vi "Calculate Center.vi"(8 "Type of Assembly Tray":i32, 9 "Syringe Coordinates":dbl[](array[numeric]), 10 "Relative Coordinates":dbl[][](array[numeric]), 11 "Fiducial Measurements":dbl[][](array[numeric])) -> (3 "XYZTheta Centers":dbl[][](array[numeric]) format="%#.9g")   [LabVIEW 2021, in "Assembly Tray.lvclass"]
uses:
  Assembly Tray.lvclass
  <vilib>/Analysis/NI_AALPro.lvlib
  <vilib>/Analysis/coordinate.llb/2D Cartesian Coordinate Rotation (Scalar).vi
panel:
  out "gantry vs OGP XY":dbl[][][](array[numeric])
  out "actual rotation":dbl[](array[numeric])
  out "Fitted relative XY coordinates":dbl[][][](array[numeric]) format="%#.6g"
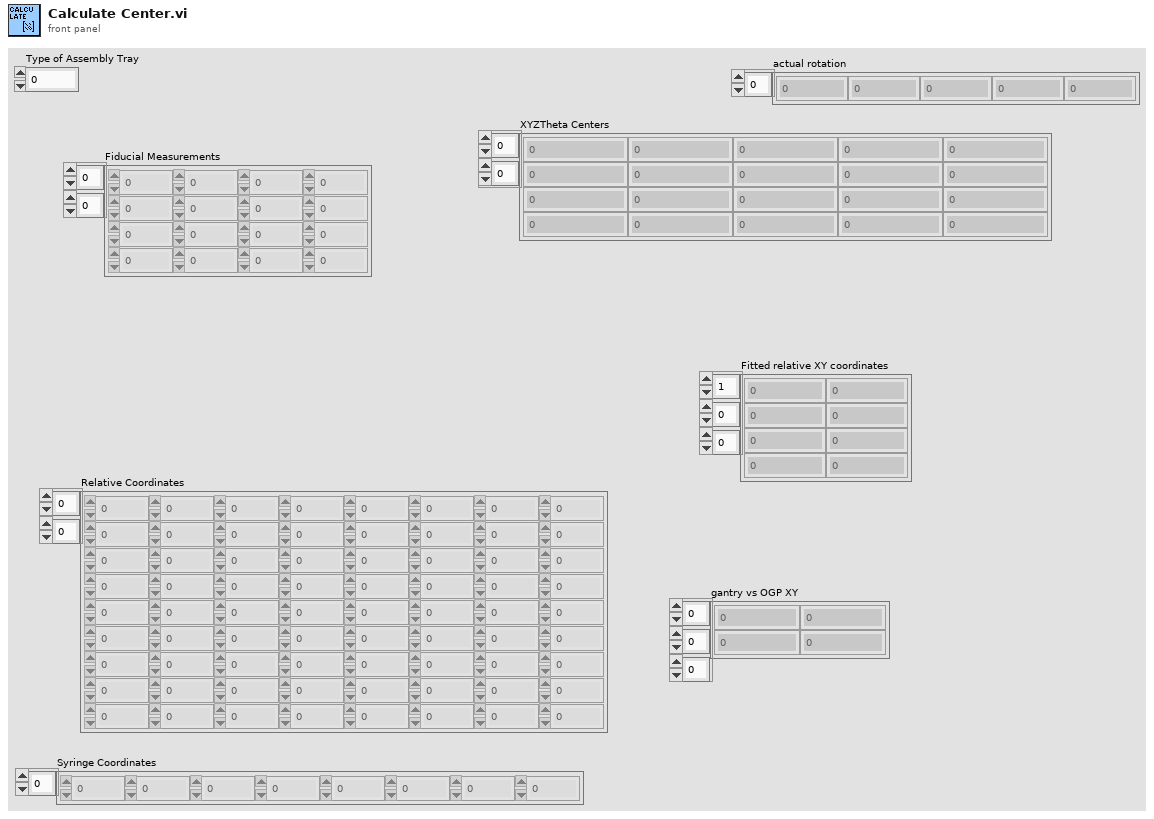
[diagram p1: front panel]
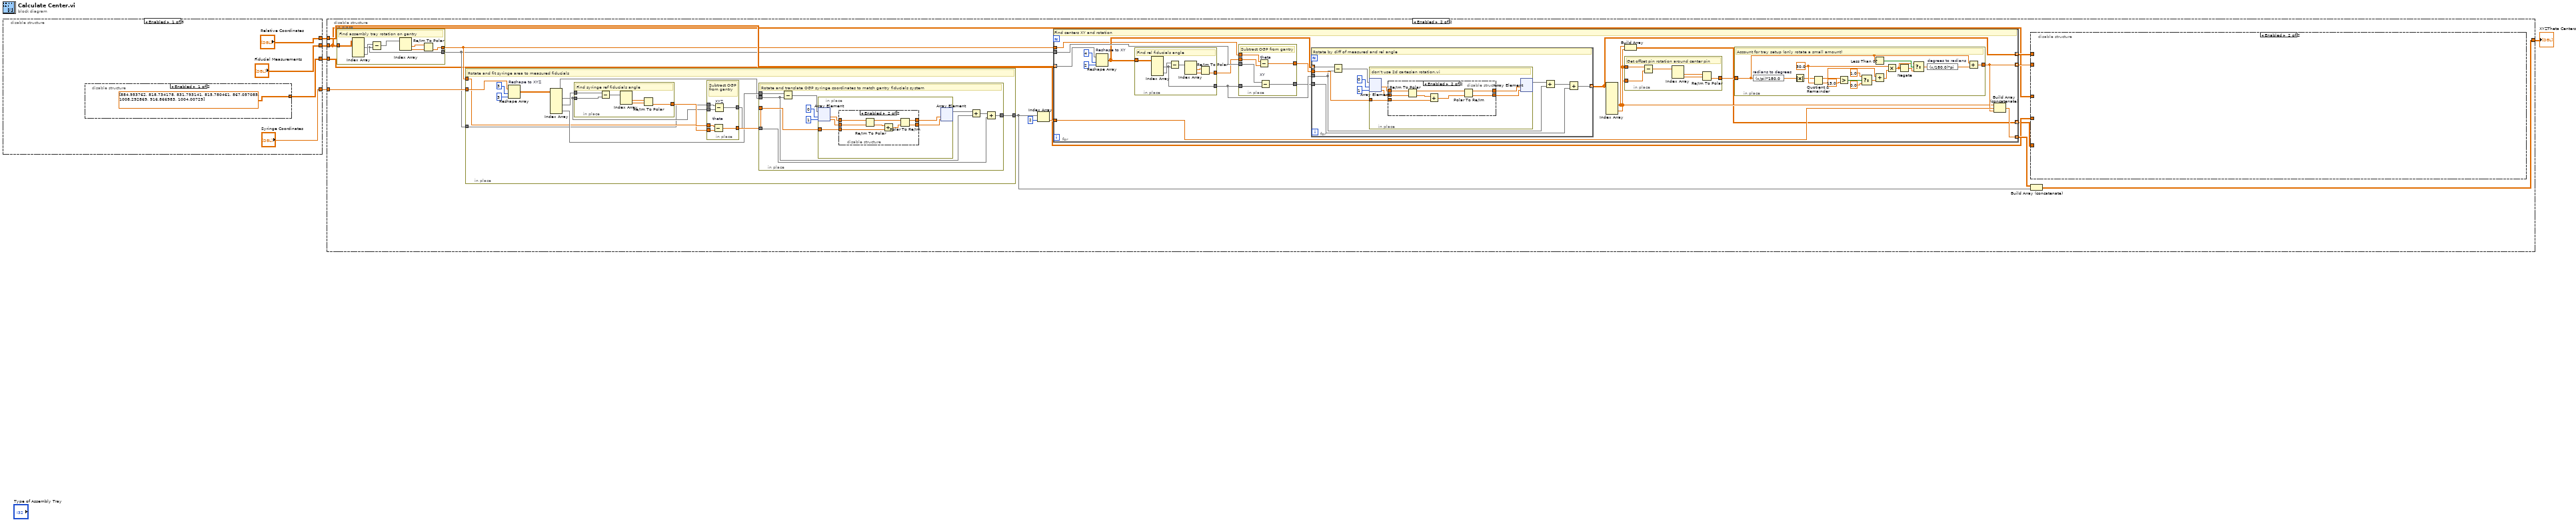
[diagram p0: block diagram]
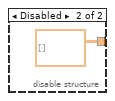
[diagram p2: hidden frame]
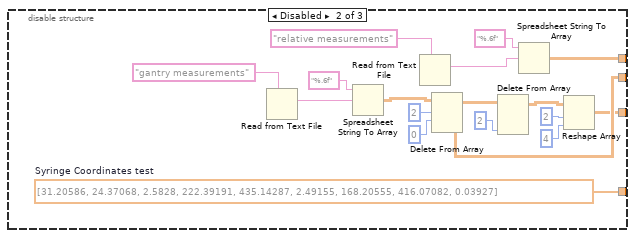
[diagram p3: hidden frame]
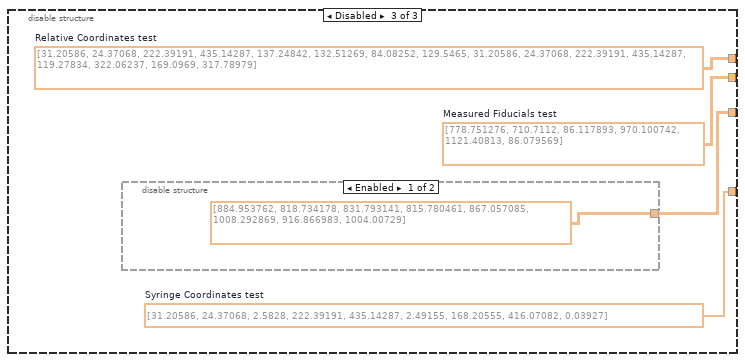
[diagram p4: hidden frame]
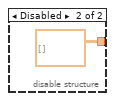
[diagram p5: hidden frame]
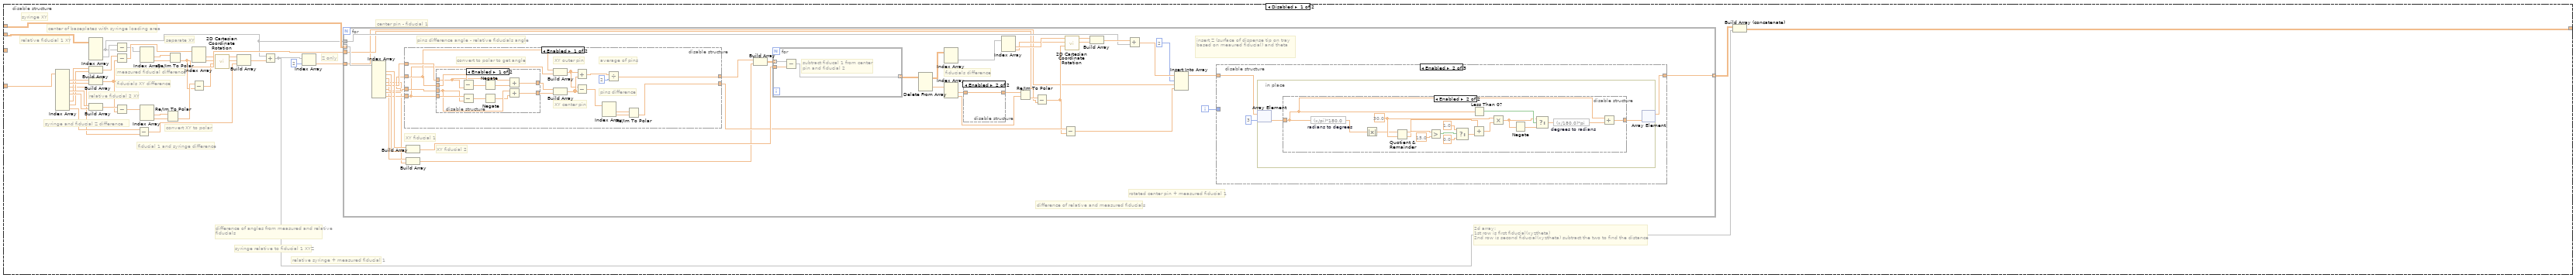
[diagram p6: hidden frame]
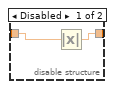
[diagram p7: hidden frame]
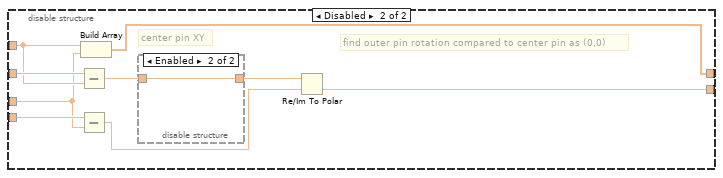
[diagram p9: hidden frame]
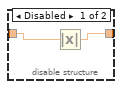
[diagram p10: hidden frame]
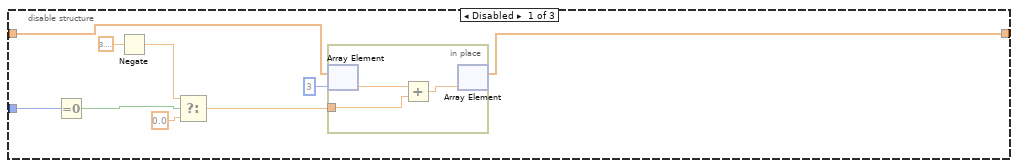
[diagram p11: hidden frame]
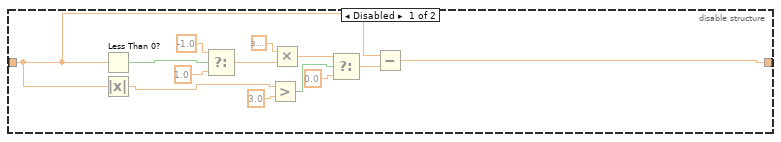
[diagram p12: hidden frame]
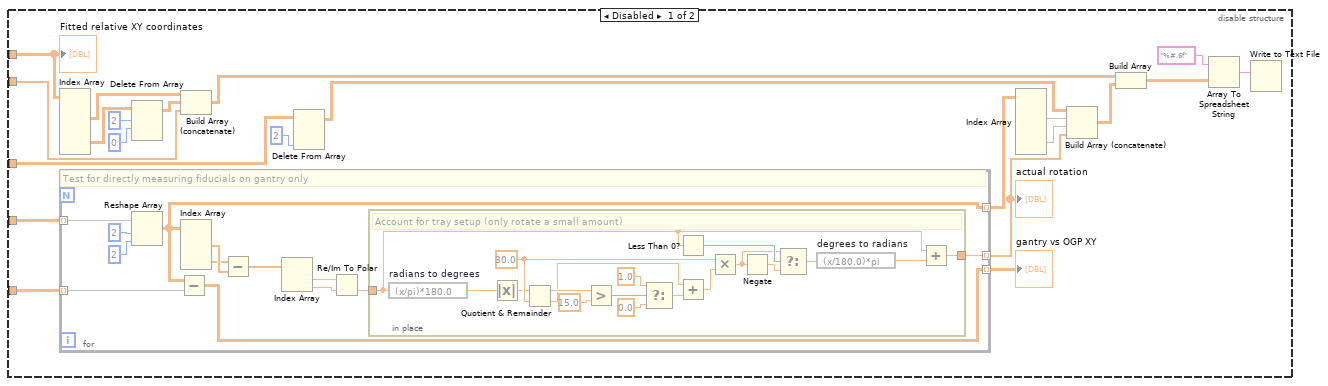
[diagram p14: hidden frame]
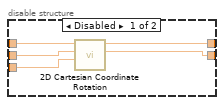
[diagram p15: hidden frame]
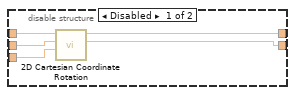
[diagram p16: hidden frame]
diagram:
  n1 = disable-structure shown="Enabled" {
    disable-tunnel: ["Syringe Coordinates" w29 w31] -> w2
    disable-tunnel: ["Fiducial Measurements" w19 w32] -> w3
    disable-tunnel: ["Relative Coordinates" w20 w33] -> w4
    disable-tunnel: [w6 w14 w30] -> w1
    frame Enabled {
      n2 = disable-structure shown="Enabled" {
        disable-tunnel: [dbl[][] [[884.953762, 818.734178, 831.793141, 815.780461], [867.057085, 1008.292869, 916.866983, 1004.00729]] dbl[][] []] -> w6
        frame Enabled {
        }
        frame Disabled {
        }
      }
    }
    frame Disabled {
      w29 = dbl[] [31.20586, 24.37068, 2.5828, 222.39191, 435.14287, 2.49155, 168.20555, 416.07082, 0.03927]  # Syringe Coordinates test
      n3 = Read from Text File(prompt (Open existing file)="gantry measurements") -> (text=w28:string)  [unwired: 3 in, 3 out]
      n4 = Spreadsheet String To Array(format string="%.6f", spreadsheet string=w28) -> (array=w12:dbl[][])  [unwired: 2 in]
      n5 = Read from Text File(prompt (Open existing file)="relative measurements") -> (text=w23:string)  [unwired: 3 in, 3 out]
      n6 = Delete From Array(array=w12, length=2, index (row)=0) -> (deleted portion=w19:dbl[][], array with subset deleted=w13:dbl[][])  [unwired: 1 in]
      n7 = Delete From Array(array=w13, index (col)=2 ("disabled index (col)")) -> (array with subset deleted=w17:dbl[][])  [unwired: 2 in, 1 out]
      n8 = Spreadsheet String To Array(format string="%.6f", spreadsheet string=w23) -> (array=w20:dbl[][])  [unwired: 2 in]
      n9 = Reshape Array(w17, 2 ("dimension size"), 4 ("dimension size")) -> (w14:dbl[][])
    }
    frame Disabled {
      w31 = dbl[] [31.20586, 24.37068, 2.5828, 222.39191, 435.14287, 2.49155, 168.20555, 416.07082, 0.03927]  # Syringe Coordinates test
      w32 = dbl[][] [[778.751276, 710.7112, 86.117893], [970.100742, 1121.40813, 86.079569]]  # Measured Fiducials test
      w33 = dbl[][] [[31.20586, 24.37068, 222.39191, 435.14287, 137.24842, 132.51269, 84.08252, 129.5465], [31.20586, 24.37068, 222.39191, 435.14287, 119.27834, 322.06237, 169.0969, 317.78979]]  # Relative Coordinates test
      n10 = disable-structure shown="Enabled" {
        disable-tunnel: [dbl[][] [[884.953762, 818.734178, 831.793141, 815.780461], [867.057085, 1008.292869, 916.866983, 1004.00729]] dbl[][] []] -> w30
        frame Enabled {
        }
        frame Disabled {
        }
      }
    }
  }
  n11 = disable-structure shown="Enabled" {
    disable-tunnel: w4 -> [w72 w217]
    disable-tunnel: w3 -> [w69 w206]
    disable-tunnel: w2 -> [w68 w216]
    disable-tunnel: [w44 w210] -> w5
    disable-tunnel: w1 -> [_ w209]
    frame Disabled {
      # "center of baseplates with syringe loading area"
      # "relative fiducial 2 XY"
      # "relative fiducial 1 XY"
      # "syringe XY"
      # "center pin - fiducial 1"
      # "Z only"
      # "relative syringe + measured fiducial 1"
      # "syringe relative to fiducial 1 XYZ"
      # "difference of angles from measured and relative fiducials"
      # "separate XY"
      # "convert XY to polar"
      # "measured fiducial difference"
      # "fiducial 1 and syringe difference"
      # "syringe and fiducial Z difference"
      # "fiducials XY difference"
      # "2d array:\n1st row is first fiducial(xyztheta)\n2nd row is second fiducial(xyztheta) subtract the two to find the distance"
      n12 = Index Array(array=w68) -> (element #1=w67:dbl, element #2=w66:dbl, element #3=w48:dbl, element #4=w64:dbl, element #5=w63:dbl, element #7=w51:dbl, element #8=w50:dbl, element #9=w49:dbl)  [unwired: 9 in, 1 out]
      n13 = Index Array(array=w69) -> (element #1=w36:dbl[], element #2=w38:dbl[])  [unwired: 4 in]
      n14 = Build Array(w51, w50) -> (w56:dbl[])
      n15 = Build Array(w67, w66) -> (w55:dbl[])
      n16 = Build Array(w64, w63) -> (w65:dbl[])
      n17 = Subtract(x=w38, y=w36) -> (x-y=w43:dbl[])
      n18 = Subtract(x=w56, y=w55) -> (x-y=w54:dbl[])
      n19 = Subtract(x=w65, y=w55) -> (x-y=w62:dbl[])
      n20 = Subtract(x=w49, y=w48) -> (x-y=w40:dbl)
      n21 = Index Array(array=w62) -> (element #1=w61:dbl, element #2=w60:dbl)  [unwired: 2 in]
      n22 = Index Array(array=w43) -> (element #1=w70:dbl, element #2=w71:dbl)  [unwired: 2 in]
      n23 = Re/Im To Polar(2:w60, 3:w61) -> (0:w59:dbl)  [unwired: 1 out]
      n24 = Re/Im To Polar(2:w71, 3:w70) -> (0:w58:dbl)  [unwired: 1 out]
      n25 = Index Array(array=w54) -> (element #1=w53:dbl, element #2=w52:dbl)  [unwired: 2 in]
      n26 = Subtract(x=w59, y=w58) -> (x-y=w57:dbl)
      n27 = call-poly <vilib>:"2D Cartesian Coordinate Rotation.vi"("theta"=w57, "y"=w52, "x"=w53) -> ("y out"=w46:dbl, "x out"=w47:dbl)  [unwired: 6 in, 1 out]
      n28 = Build Array(w47, w46, w40) -> (w37:dbl[])
      n29 = Add(x=w36, y=w37) -> (x+y=w39:dbl[])
      n30 = Index Array(array=w39, index=2) -> (element=w41:dbl)
      n31 = for {
        tunnel: w72 -> [w89] mode=indexing
        tunnel: [w80] -> w45 mode=indexing
        tunnel: w36 -> [w88]
        tunnel: w58 -> [w87]
        tunnel: w41 -> [w86]
        i -> [w79]
        # "insert Z (surface of dispense tip on tray based on meaured fiducial) and theta"
        # "pins difference angle - relative fiducials angle"
        # "rotated center pin + measured fiducial 1"
        # "difference of relative and measured fiducials"
        # "fiducials difference"
        # "XY fiducial 2"
        # "XY fiducial 1"
        n32 = Index Array(array=w89) -> (element #1=w109:dbl, element #2=w108:dbl, element #3=w78:dbl, element #4=w77:dbl, element #5=w84:dbl, element #6=w85:dbl, element #7=w83:dbl, element #8=w82:dbl)  [unwired: 8 in]
        n33 = disable-structure shown="Enabled" {
          disable-tunnel: [w125 w140] -> w93
          disable-tunnel: [w119 w144] -> w91
          disable-tunnel: w85 -> [w116 w141]
          disable-tunnel: w84 -> [w115 w142]
          disable-tunnel: w83 -> [w114 w145]
          disable-tunnel: w82 -> [w113 w143]
          frame Enabled {
            # "convert to polar to get angle"
            # "pins difference"
            # "average of pins"
            # "XY outer pin"
            # "XY center pin"
            n34 = disable-structure shown="Enabled" {
              disable-tunnel: w113 -> [w137 _]
              disable-tunnel: w114 -> [w136 _]
              disable-tunnel: w116 -> [w133 w139]
              disable-tunnel: w115 -> [w130 w138]
              disable-tunnel: [w129 w139] -> w117
              disable-tunnel: [w128 w138] -> w118
              frame Enabled {
                n35 = Subtract(x=w136, y=w130) -> (x-y=w134:dbl)
                n36 = Subtract(x=w137, y=w133) -> (x-y=w135:dbl)
                n37 = Negate(x=w134) -> (-x=w131:dbl)
                n38 = Negate(x=w135) -> (-x=w132:dbl)
                n39 = Add(x=w130, y=w131) -> (x+y=w128:dbl)
                n40 = Add(x=w133, y=w132) -> (x+y=w129:dbl)
              }
              frame Disabled {
              }
            }
            n41 = Build Array(w114, w113) -> (w123:dbl[])
            n42 = Build Array(w118, w117) -> (w124:dbl[])
            n43 = Add(x=w123, y=w124) -> (x+y=w126:dbl[])
            n44 = Subtract(x=w123, y=w124) -> (x-y=w122:dbl[])
            n45 = Index Array(array=w122) -> (element #1=w121:dbl, element #2=w120:dbl)  [unwired: 2 in]
            n46 = Divide(x=w126, y=2) -> (x/y=w125:dbl[])
            n47 = Re/Im To Polar(2:w120, 3:w121) -> (0:w119:dbl)  [unwired: 1 out]
          }
          frame Disabled {
            # "find outer pin rotation compared to center pin as (0,0)"
            # "center pin XY"
            n48 = Subtract(x=w145, y=w142) -> (x-y=w147:dbl)
            n49 = Subtract(x=w143, y=w141) -> (x-y=w148:dbl)
            n50 = Build Array(w142, w141) -> (w140:dbl[])
            n51 = disable-structure shown="Enabled" {
              disable-tunnel: w147 -> [w150 w151]
              disable-tunnel: [w149 w151] -> w146
              frame Disabled {
                n52 = Absolute Value(x=w150) -> (abs(x)=w149:dbl)
              }
              frame Enabled {
              }
            }
            n53 = Re/Im To Polar(2:w148, 3:w146) -> (0:w144:dbl)  [unwired: 1 out]
          }
        }
        n54 = Build Array(w109, w108) -> (w106:dbl[])
        n55 = Build Array(w78, w77) -> (w76:dbl[])
        n56 = Build Array(w93, w76) -> (w107:dbl[][])
        n57 = for {
          tunnel: w107 -> [w203] mode=indexing
          tunnel: w106 -> [w202]
          tunnel: [w201] -> w105 mode=indexing
          # "subtract fiducal 1 from center pin and fiducial 2"
          n58 = Subtract(x=w203, y=w202) -> (x-y=w201:dbl[])
        }
        n59 = Delete From Array(array=w105) -> (deleted portion=w104:dbl[], array with subset deleted=w102:dbl[][])  [unwired: 3 in]
        n60 = Index Array(array=w102) -> (element=w101:dbl[])  [unwired: 2 in]
        n61 = Index Array(array=w104) -> (element #1=w75:dbl, element #2=w103:dbl)  [unwired: 2 in]
        n62 = disable-structure shown="Enabled" {
          disable-tunnel: w75 -> [w111 w112]
          disable-tunnel: [w110 w112] -> w74
          frame Disabled {
            n63 = Absolute Value(x=w111) -> (abs(x)=w110:dbl)
          }
          frame Enabled {
          }
        }
        n64 = Index Array(array=w101) -> (element #1=w100:dbl, element #2=w99:dbl)  [unwired: 2 in]
        n65 = Re/Im To Polar(2:w103, 3:w74) -> (0:w92:dbl)  [unwired: 1 out]
        n66 = Subtract(x=w92, y=w87) -> (x-y=w90:dbl)
        n67 = Subtract(x=w91, y=w90) -> (x-y=w73:dbl)
        n68 = call-poly <vilib>:"2D Cartesian Coordinate Rotation.vi"("theta"=w90, "y"=w99, "x"=w100) -> ("y out"=w96:dbl, "x out"=w97:dbl)  [unwired: 6 in, 1 out]
        n69 = Build Array(w97, w96) -> (w98:dbl[])
        n70 = Add(x=w98, y=w88) -> (x+y=w95:dbl[])
        n71 = Insert Into Array(array=w95, index=2, new element #1=w86, new element #2=w73) -> (w81:dbl[])
        n72 = disable-structure shown="Enabled" {
          disable-tunnel: w81 -> [w160 w166 w200]
          disable-tunnel: [w159 w165 w200] -> w80
          disable-tunnel: w79 -> [w157 _ _]
          frame Disabled {
            n73 = Equal To 0?(x=w157) -> (x = 0?=w155:bool)
            n74 = Negate(x=3.141592653589793) -> (-x=w152:dbl)
            n75 = Select(t=w152, s=w155, f=0.0) -> (s? t:f=w154:dbl)
            n76 = in-place {
              in-place-border: w154 -> [w161]
              n77 = in-place-array #1(w160, 3) -> (w163:dbl)
              n78 = Add(x=w163, y=w161) -> (x+y=w162:dbl)
              n79 = in-place-array #1(w162) -> (w159:dbl[])  [unwired: 1 out]
            }
          }
          frame Enabled {
            n80 = in-place {
              n81 = in-place-array #2(w166, 3) -> (w168:dbl)
              n82 = disable-structure shown="Enabled" {
                disable-tunnel: w168 -> [w175 w185]
                disable-tunnel: [w174 w184] -> w167
                frame Disabled {
                  n83 = Less Than 0?(x=w175) -> (x < 0?=w181:bool)
                  n84 = Absolute Value(x=w175) -> (abs(x)=w178:dbl)
                  n85 = Select(t=-1.0, s=w181, f=1.0) -> (s? t:f=w170:dbl)
                  n86 = Greater?(x=w178, y=3.0) -> (0:w176:bool)
                  n87 = Multiply(x=3.141592653589793, y=w170) -> (x*y=w169:dbl)
                  n88 = Select(t=w169, s=w176, f=0.0) -> (s? t:f=w172:dbl)
                  n89 = Subtract(x=w175, y=w172) -> (x-y=w174:dbl)
                }
                frame Enabled {
                  w192 = 30.0 ("y")
                  n90 = expression code="(x/pi)*180.0" "radians to degrees"(w185) -> (w183:dbl)
                  n91 = Absolute Value(x=w183) -> (abs(x)=w182:dbl)
                  n92 = Quotient & Remainder(x=w182, y=w192) -> (x-y*floor(x/y)=w199:dbl, floor(x/y)=w193:dbl)
                  n93 = Greater?(x=w199, y=15.0) -> (0:w197:bool)
                  n94 = Select(t=1.0, s=w197, f=0.0) -> (s? t:f=w194:dbl)
                  n95 = Add(x=w193, y=w194) -> (x+y=w191:dbl)
                  n96 = Less Than 0?(x=w185) -> (x < 0?=w190:bool)
                  n97 = Multiply(x=w192, y=w191) -> (x*y=w189:dbl)
                  n98 = Negate(x=w189) -> (-x=w188:dbl)
                  n99 = Select(t=w189, s=w190, f=w188) -> (s? t:f=w187:dbl)
                  n100 = expression code="(x/180.0)*pi" "degrees to radians"(w187) -> (w186:dbl)
                  n101 = Add(x=w185, y=w186) -> (x+y=w184:dbl)
                }
              }
              n102 = in-place-array #2(w167) -> (w165:dbl[])  [unwired: 1 out]
            }
          }
          frame Disabled {
          }
        }
      }
      n103 = Build Array (concatenate)(w45, w39) -> (w44:dbl[][])
    }
    frame Enabled {
      n104 = in-place {
        in-place-border: w206 -> [w407]
        in-place-border: [w411] -> w215
        in-place-border: [w408] -> w214
        # "Find assembly tray rotation on gantry"
        n105 = Index Array(array=w407) -> (element #1=w408:dbl[], element #2=w409:dbl[])  [unwired: 4 in]
        n106 = Subtract(x=w409, y=w408) -> (x-y=w410:dbl[])
        n107 = Index Array(array=w410) -> (element #1=w412:dbl, element #2=w413:dbl)  [unwired: 2 in]
        n108 = Re/Im To Polar(2:w413, 3:w412) -> (0:w411:dbl)  [unwired: 1 out]
      }
      n109 = in-place {
        in-place-border: w216 -> [w283]
        in-place-border: w215 -> [w276]
        in-place-border: w214 -> [w273]
        in-place-border: [w271] -> w204
        # "Rotate and fit syringe area to measured fiducials"
        n110 = Reshape Array "Reshape to XYZ"(w283, 3 ("dimension size"), 3 ("dimension size")) -> (w279:dbl[][])
        n111 = Index Array(array=w279) -> (element #1=w274:dbl[], element #2=w278:dbl[], element #3=w277:dbl[])  [unwired: 6 in]
        n112 = in-place {
          in-place-border: [w320] -> w275
          in-place-border: w274 -> [w319]
          in-place-border: w278 -> [w318]
          # "Find syringe ref fiducials angle"
          n113 = Subtract(x=w318, y=w319) -> (x-y=w321:dbl[])
          n114 = Index Array(array=w321) -> (element #1=w322:dbl, element #2=w323:dbl)  [unwired: 2 in]
          n115 = Re/Im To Polar(2:w323, 3:w322) -> (0:w320:dbl)  [unwired: 1 out]
        }
        n116 = in-place {
          in-place-border: [w289] -> w280
          in-place-border: w276 -> [w288]
          in-place-border: w275 -> [w287]
          in-place-border: w274 -> [w286]
          in-place-border: w273 -> [w285]
          in-place-border: [w284] -> w272
          # "Subtract OGP from gantry"
          n117 = Subtract "theta"(x=w288, y=w287) -> (x-y=w289:dbl)
          n118 = Subtract "XYZ"(x=w285, y=w286) -> (x-y=w284:dbl[])
        }
        n119 = in-place {
          in-place-border: w280 -> [w299]
          in-place-border: w277 -> [w296]
          in-place-border: w274 -> [w293]
          in-place-border: w272 -> [w292]
          in-place-border: [w290] -> w271
          # "Rotate and translate OGP syringe coordinates to match gantry fiducials system"
          n120 = Subtract(x=w296, y=w293) -> (x-y=w295:dbl[])
          n121 = in-place {
            in-place-border: w299 -> [w304]
            n122 = in-place-array #3(w295, 0, 1) -> (w303:dbl, w302:dbl)
            n123 = disable-structure shown="Enabled" {
              disable-tunnel: w304 -> [w309 w312]
              disable-tunnel: w303 -> [w308 w315]
              disable-tunnel: w302 -> [w307 w314]
              disable-tunnel: [w306 w317] -> w301
              disable-tunnel: [w305 w316] -> w300
              frame Disabled {
                n124 = call-poly <vilib>:"2D Cartesian Coordinate Rotation.vi"("theta"=w309, "y"=w307, "x"=w308) -> ("y out"=w305:dbl, "x out"=w306:dbl)  [unwired: 6 in, 1 out]
              }
              frame Enabled {
                n125 = Re/Im To Polar(2:w314, 3:w315) -> (0:w313:dbl, 1:w311:dbl)
                n126 = Add(x=w313, y=w312) -> (x+y=w310:dbl)
                n127 = Polar To Re/Im(2:w310, 3:w311) -> (0:w316:dbl, 1:w317:dbl)
              }
            }
            n128 = in-place-array #3(w301, w300) -> (w294:dbl[])  [unwired: 2 out]
          }
          n129 = Add(x=w294, y=w293) -> (x+y=w291:dbl[])
          n130 = Add(x=w291, y=w292) -> (x+y=w290:dbl[])
        }
      }
      n131 = Index Array(array=w204, index=2) -> (element=w212:dbl)
      n132 = for {
        tunnel: w217 -> [w341] mode=indexing
        tunnel: w215 -> [w326]
        tunnel: w214 -> [w338]
        tunnel: [w327] -> w208 mode=indexing
        tunnel: [w337] -> w211 mode=indexing
        tunnel: w212 -> [w336]
        tunnel: [w334] -> w207 mode=indexing
        tunnel: [w329] -> w205 mode=indexing
        # "Find centers XY and rotation"
        n133 = Reshape Array "Reshape to XY"(w341, 4 ("dimension size"), 2 ("dimension size")) -> (w332:dbl[][])
        n134 = in-place {
          in-place-border: [w356] -> w325
          in-place-border: w332 -> [w355]
          in-place-border: [w354] -> w333
          # "Find rel fiducials angle"
          n135 = Index Array(array=w355) -> (element #1=w354:dbl[], element #2=w360:dbl[])  [unwired: 4 in]
          n136 = Subtract(x=w360, y=w354) -> (x-y=w357:dbl[])
          n137 = Index Array(array=w357) -> (element #1=w358:dbl, element #2=w359:dbl)  [unwired: 2 in]
          n138 = Re/Im To Polar(2:w359, 3:w358) -> (0:w356:dbl)  [unwired: 1 out]
        }
        n139 = in-place {
          in-place-border: [w347] -> w328
          in-place-border: w338 -> [w346]
          in-place-border: w333 -> [w345]
          in-place-border: w326 -> [w343]
          in-place-border: w325 -> [w342]
          in-place-border: [w344] -> w324
          # "Subtract OGP from gantry"
          n140 = Subtract "theta"(x=w343, y=w342) -> (x-y=w344:dbl)
          n141 = Subtract "XY"(x=w346, y=w345) -> (x-y=w347:dbl[])
        }
        n142 = for {
          tunnel: w324 -> [w388]
          tunnel: w332 -> [w387] mode=indexing
          tunnel: w333 -> [w382]
          tunnel: w328 -> [w380]
          tunnel: [w379] -> w327 mode=indexing
          # "Rotate by diff of measured and rel angle"
          n143 = Subtract(x=w387, y=w382) -> (x-y=w386:dbl[])
          n144 = in-place {
            in-place-border: w388 -> [w393]
            # "don't use 2d cartesian rotation.vi"
            n145 = in-place-array #4(w386, 0, 1) -> (w390:dbl, w389:dbl)
            n146 = disable-structure shown="Enabled" {
              disable-tunnel: w393 -> [w398 w401]
              disable-tunnel: [w397 w400] -> w392
              disable-tunnel: [w396 w399] -> w391
              disable-tunnel: w390 -> [w395 w403]
              disable-tunnel: w389 -> [w394 w402]
              frame Disabled {
                n147 = call-poly <vilib>:"2D Cartesian Coordinate Rotation.vi"("theta"=w398, "y"=w394, "x"=w395) -> ("y out"=w396:dbl, "x out"=w397:dbl)  [unwired: 6 in, 1 out]
              }
              frame Enabled {
                n148 = Re/Im To Polar(2:w402, 3:w403) -> (0:w406:dbl, 1:w405:dbl)
                n149 = Add(x=w406, y=w401) -> (x+y=w404:dbl)
                n150 = Polar To Re/Im(2:w404, 3:w405) -> (0:w399:dbl, 1:w400:dbl)
              }
            }
            n151 = in-place-array #4(w392, w391) -> (w383:dbl[])  [unwired: 2 out]
          }
          n152 = Add(x=w383, y=w382) -> (x+y=w381:dbl[])
          n153 = Add(x=w381, y=w380) -> (x+y=w379:dbl[])
        }
        n154 = Index Array(array=w327) -> (element #3=w331:dbl[], element #4=w330:dbl[])  [unwired: 8 in, 2 out]
        n155 = Build Array(w331, w330) -> (w329:dbl[][])
        n156 = in-place {
          in-place-border: w330 -> [w353]
          in-place-border: [w349] -> w335
          in-place-border: w331 -> [w348]
          # "Get offset pin rotation around center pin"
          n157 = Subtract(x=w353, y=w348) -> (x-y=w352:dbl[])
          n158 = Index Array(array=w352) -> (element #1=w351:dbl, element #2=w350:dbl)  [unwired: 2 in]
          n159 = Re/Im To Polar(2:w350, 3:w351) -> (0:w349:dbl)  [unwired: 1 out]
        }
        n160 = in-place {
          in-place-border: [w361] -> w334
          in-place-border: w335 -> [w362]
          w371 = 30.0 ("y")
          # "Account for tray setup (only rotate a small amount)"
          n161 = expression code="(x/pi)*180.0" "radians to degrees"(w362) -> (w364:dbl)
          n162 = Absolute Value(x=w364) -> (abs(x)=w363:dbl)
          n163 = Quotient & Remainder(x=w363, y=w371) -> (x-y*floor(x/y)=w378:dbl, floor(x/y)=w372:dbl)
          n164 = Greater?(x=w378, y=15.0) -> (0:w376:bool)
          n165 = Select(t=1.0, s=w376, f=0.0) -> (s? t:f=w373:dbl)
          n166 = Less Than 0?(x=w362) -> (x < 0?=w369:bool)
          n167 = Add(x=w372, y=w373) -> (x+y=w370:dbl)
          n168 = Multiply(x=w371, y=w370) -> (x*y=w368:dbl)
          n169 = Negate(x=w368) -> (-x=w367:dbl)
          n170 = Select(t=w368, s=w369, f=w367) -> (s? t:f=w366:dbl)
          n171 = expression code="(x/180.0)*pi" "degrees to radians"(w366) -> (w365:dbl)
          n172 = Add(x=w362, y=w365) -> (x+y=w361:dbl)
        }
        n173 = Build Array (concatenate)(w331, w336, w334) -> (w337:dbl[])
      }
      n174 = disable-structure shown="Enabled" {
        disable-tunnel: w209 -> [w229 _]
        disable-tunnel: w208 -> [w227 _]
        disable-tunnel: w207 -> [w231 _]
        disable-tunnel: w206 -> [w222 _]
        disable-tunnel: w205 -> [w218 _]
        frame Disabled {
          n175 = Index Array(array=w227) -> (element #1=w234:dbl[][], element #2=w225:dbl[][])  [unwired: 6 in]
          n176 = for {
            tunnel: w229 -> [w243] mode=indexing
            tunnel: [w249] -> w237 mode=indexing
            tunnel: [w242] -> w228 mode=indexing
            tunnel: w218 -> [w241] mode=indexing
            tunnel: [w240] -> w226 mode=indexing
            # "Test for directly measuring fiducials on gantry only"
            n177 = Reshape Array(w243, 2 ("dimension size"), 2 ("dimension size")) -> (w242:dbl[][])
            n178 = Subtract(x=w242, y=w241) -> (x-y=w240:dbl[][])
            n179 = Index Array(array=w242) -> (element #1=w248:dbl[], element #2=w247:dbl[])  [unwired: 4 in]
            n180 = Subtract(x=w247, y=w248) -> (x-y=w246:dbl[])
            n181 = Index Array(array=w246) -> (element #1=w252:dbl, element #2=w251:dbl)  [unwired: 2 in]
            n182 = Re/Im To Polar(2:w251, 3:w252) -> (0:w250:dbl)  [unwired: 1 out]
            n183 = in-place {
              in-place-border: [w253] -> w249
              in-place-border: w250 -> [w254]
              w263 = 30.0 ("y")
              # "Account for tray setup (only rotate a small amount)"
              n184 = expression code="(x/pi)*180.0" "radians to degrees"(w254) -> (w256:dbl)
              n185 = Absolute Value(x=w256) -> (abs(x)=w255:dbl)
              n186 = Quotient & Remainder(x=w255, y=w263) -> (x-y*floor(x/y)=w270:dbl, floor(x/y)=w264:dbl)
              n187 = Greater?(x=w270, y=15.0) -> (0:w268:bool)
              n188 = Select(t=1.0, s=w268, f=0.0) -> (s? t:f=w265:dbl)
              n189 = Less Than 0?(x=w254) -> (x < 0?=w261:bool)
              n190 = Add(x=w264, y=w265) -> (x+y=w262:dbl)
              n191 = Multiply(x=w263, y=w262) -> (x*y=w260:dbl)
              n192 = Negate(x=w260) -> (-x=w259:dbl)
              n193 = Select(t=w260, s=w261, f=w259) -> (s? t:f=w258:dbl)
              n194 = expression code="(x/180.0)*pi" "degrees to radians"(w258) -> (w257:dbl)
              n195 = Add(x=w254, y=w257) -> (x+y=w253:dbl)
            }
          }
          "actual rotation" <- w237
          "gantry vs OGP XY" <- w226
          n196 = Delete From Array(array=w225, length=2, index (row)=0) -> (array with subset deleted=w219:dbl[][])  [unwired: 1 in, 1 out]
          n197 = Build Array (concatenate)(w234, w219, w231) -> (w235:dbl[][])
          n198 = Delete From Array(array=w222, index (col)=2 ("disabled index (col)")) -> (array with subset deleted=w220:dbl[][])  [unwired: 2 in, 1 out]
          n199 = Index Array(array=w228) -> (element #1=w239:dbl[][], element #2=w238:dbl[][])  [unwired: 6 in]
          n200 = Build Array (concatenate)(w220, w239, w238, w237) -> (w232:dbl[][])
          n201 = Build Array(w235, w232) -> (w236:dbl[][][])
          n202 = Array To Spreadsheet String(array=w236, 3:"%#.6f" ("format string")) -> (spreadsheet string=w233:string)  [unwired: 1 in]
          n203 = Write to Text File(text=w233) -> ()  [unwired: 3 in, 3 out]
          "Fitted relative XY coordinates" <- w227
        }
        frame Enabled {
        }
      }
      n204 = Build Array (concatenate)(w211, w204) -> (w210:dbl[][])
    }
  }
  "XYZTheta Centers" <- w5
